vi "VIH - CHM Project - Write Info File.vi"(7 "Expect HHP exist (T)":bool=TRUE, 8 "error in":errorcluster, 10 "HHP_Generation":T1={"HHP_Template"=enum."default", "HHP_Template_CustomPath"=path "", "HHP_Target"=enum."default", "HHP_Target_CustomPath"=path "", "HHP_CreateTOC"=TRUE, "HHP_CreateIDX"=TRUE, "HHP_DefaultTopic"=enum."auto", "HHP_DefaultTopic_CustomPath"=path "", "CHM_Filename"=path "", "HHP_AutoBuild"=FALSE, "CHM_AutoBuild"=FALSE}, 11 "Project Tree":T2) -> (0 "error out":errorcluster, 1 "Info File":path, 2 "Target HHP File":path, 3 "dup Project Tree":T2)   [LabVIEW 2014]
doc: "::: VI Helpeks :::\nCopyright (c) 2000-2026 Konstantin Shifershteyn. All rights reserved."
uses:
  _VIH Project Manager.llb/VIH Project Tree Typedef - Tree Refnum.ctl
  VIH - CHM Project - HHP Generation Params Cluster.ctl
panel:
  # "VI Helpeks\nCopyright (c) 2012-2026 Konstantin Shifershteyn"
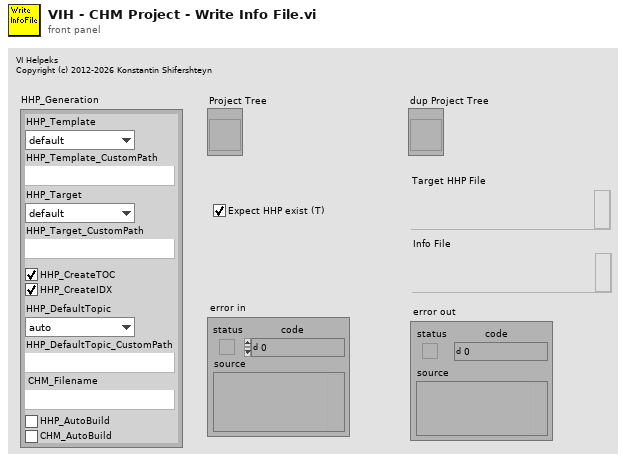
[diagram p1: front panel]
types:
  T1 = typedef "VIH - CHM Project - HHP Generation Params Cluster.ctl" = cluster{"HHP_Template":enum16{"default", "custom"}, "HHP_Template_CustomPath":path, "HHP_Target":enum16{"default", "custom"}, "HHP_Target_CustomPath":path, "HHP_CreateTOC":bool, "HHP_CreateIDX":bool, "HHP_DefaultTopic":enum16{"auto", "custom"}, "HHP_DefaultTopic_CustomPath":path, "CHM_Filename":path, "HHP_AutoBuild":bool, "CHM_AutoBuild":bool}
  T2 = typedef "VIH Project Tree Typedef - Tree Refnum.ctl" = refnum<vi>
  T3 = enum16{"nop", "Init", "Run-HHP", "Run-CHM", "Run-INFO"}
  T4 = cluster{"TOC File":path, "IDX File":path, "HTML Files":path[], "Default Topic File":path, "Compiled File":path}
  T5 = typedef "VIH HelpGen Typedef - Palette - Item Type Enum.ctl" = enum32{"<Invalid>", "<unknown>", "VI", "Menu", "LV Func", "Express VI", "Poly VI", "CTL", "HTML"}
  T6 = cluster{"Types":T5[], "Src Paths":path[], "Dynamic":enum16{"Dyn", "Stat", "Both"}[], "HTML Paths":path[], "HTML Titles":string[]}
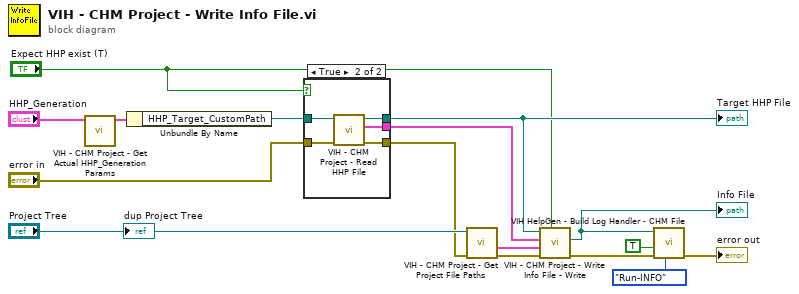
[diagram p0: block diagram]
diagram:
  n1 = call "VIH - CHM Project - Get Actual HHP_Generation Params.vi"("HHP_Generation"="HHP_Generation") -> ("HHP_Generation out"=w13:T1)  [unwired: 8 in, 2 out]
  n2 = Unbundle By Name(w13) -> ("HHP_Target_CustomPath"=w8:path)
  n3 = case shown="True" "Expect HHP exist (T)" {
    tunnel: [w17 w23] -> w14
    tunnel: "error in" -> [w17 w22]
    tunnel: [_ w21] -> w9
    tunnel: w8 -> [w18 w20]
    tunnel: [w18 w19] -> w7
    frame False {
    }
    frame True {
      n4 = call "VIH - CHM Project - Read HHP File.vi"("error in"=w22, "HHP File"=w20) -> ("error out"=w23:errorcluster, "Files"=w21:T4, "dup HHP File"=w19:path)  [unwired: 7 in]
    }
  }
  "Target HHP File" <- w7
  n5 = call "VIH - CHM Project - Get Project File Paths.vi"("error in"=w14, "Project Tree"="Project Tree") -> ("error out"=w11:errorcluster, "Project Files"=w10:T6)  [unwired: 7 in, 1 out]
  n6 = call "VIH - CHM Project - Write Info File - Write.vi"("Expect HHP exist (T)"="Expect HHP exist (T)", "error in"=w11, "Project Files"=w10, "Files in HHP"=w9, "Target HHP File"=w7) -> ("error out"=w5:errorcluster, "Info File"=w4:path)  [unwired: 5 in]
  "Info File" <- w4
  n7 = call "VIH HelpGen - Build Log Handler - CHM File.vi"("cmd (nop)"=T3."Run-INFO", "error in"=w5, "File Built"=TRUE, "File Path 1"=w4) -> ("error out"=→"error out":errorcluster)  [unwired: 5 in, 2 out]
  "dup Project Tree" <- "Project Tree"
